vi "Add Files to Project.vi"(8 "error in":errorcluster, 11 "Runner in":refnum<class "Runner.lvclass">) -> (0 "error out":errorcluster, 3 "Runner out":refnum<class "Runner.lvclass">)   [LabVIEW 2026, in "Runner.lvlib" / "Runner.lvclass"]
doc: "This method adds all created files (VIs and Type Definitions) to the project."
uses:
  Runner.lvclass
  Runner.lvclass/Runner.ctl
  Interfaces/ILogger/ILogger Messages/Log Msg/Log Msg.lvclass/Log Msg.ctl
  <vilib>/ActorFramework/Message Enqueuer/Message Enqueuer.lvclass/Message Enqueuer.ctl
  <vilib>/ActorFramework/Message Enqueuer/Enqueue.vi
  Interfaces/ILogger/ILogger Messages/Log Msg/Log Msg.lvclass
  <userlib>/_OpenG.lib/file/file.llb/File Exists - Scalar__ogtk.vi
  <vilib>/ActorFramework/Message Priority Queue/Priority Enqueue.vi
  Interfaces/IProject Manager/IProject Manager.lvclass
  <userlib>/_OpenG.lib/file/file.llb/openg_file.lvlib
  Interfaces/IFile Manager/IFile Manager.lvclass
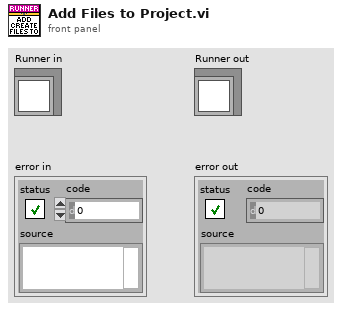
[diagram p1: front panel]
types:
  T1 = typedef "Log Entry--cluster.ctl" = cluster{"Time":timestamp, "Message":string}
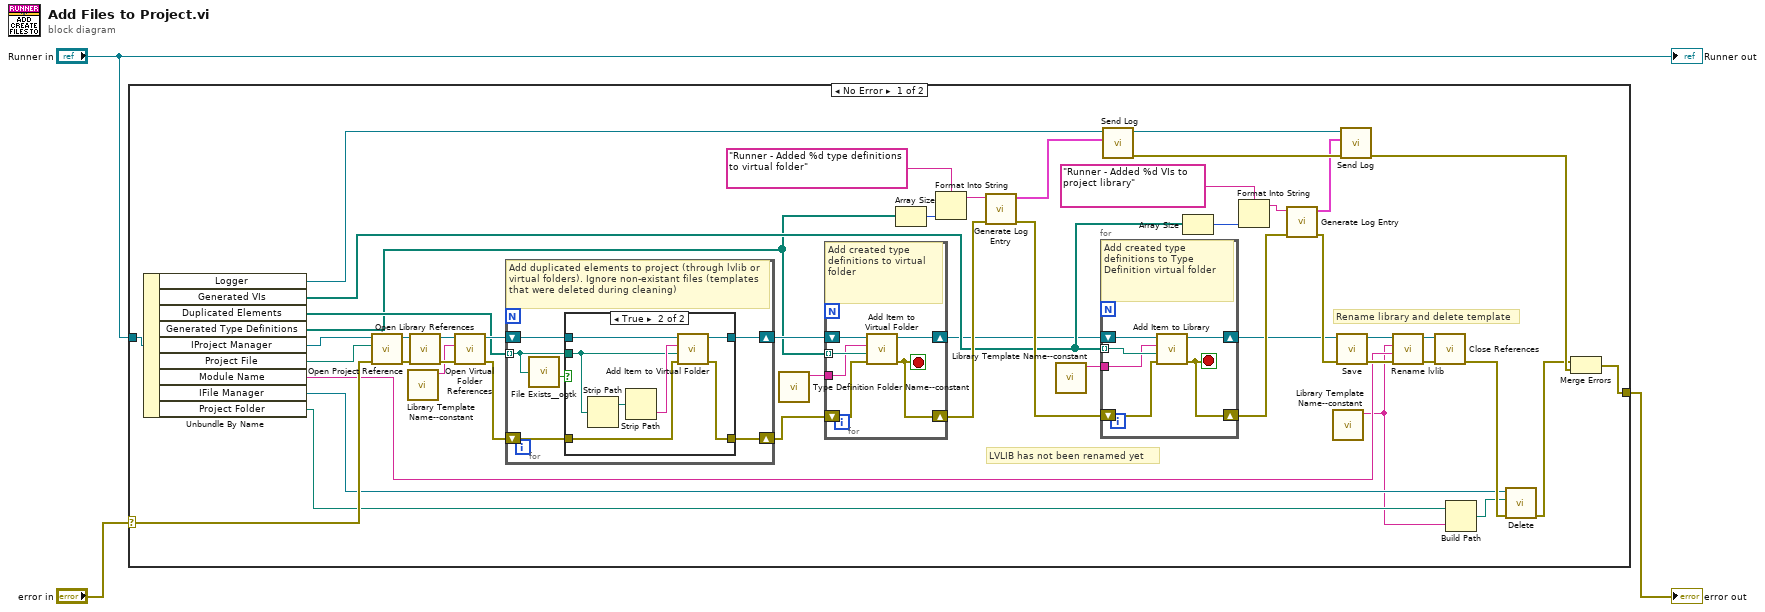
[diagram p0: block diagram]
diagram:
  n1 = case shown="No Error" "error in" {
    selector: "error in" -> [w40 w79]
    tunnel: "Runner in" -> [w35 _]
    tunnel: [w50 w79] -> w2
    frame No Error {
      # "Rename library and delete template"
      # "LVLIB has not been renamed yet"
      n2 = Unbundle By Name(w35) -> ("Logger"=w25:refnum<class "Message Enqueuer.lvclass">, "Generated VIs"=w27:path[], "Duplicated Elements"=w10:path[], "Generated Type Definitions"=w8:path[], "IProject Manager"=w14:refnum<class "IProject Manager.lvclass">, "Project File"=w12:path, "Module Name"=w13:string, "IFile Manager"=w7:refnum<class "IFile Manager.lvclass">, "Project Folder"=w6:path)
      n3 = call-dynamic "Open Project Reference.vi"("error in"=w40, "Path"=w12, "IProject Manager in"=w14) -> ("error out"=w41:errorcluster, "IProject Manager out"=w15:refnum<class "IProject Manager.lvclass">)  [unwired: 7 in]
      n4 = call "Library Template Name--constant.vi"() -> ("Library Template Name"=w17:string)  [unwired: 11 in]
      n5 = call-dynamic "Open Library References.vi"("error in"=w41, "IProject Manager in"=w15) -> ("error out"=w42:errorcluster, "IProject Manager out"=w16:refnum<class "IProject Manager.lvclass">)  [unwired: 8 in]
      n6 = call-dynamic "Open Virtual Folder References.vi"("error in"=w42, "lvlib"=w17, "IProject Manager in"=w16) -> ("error out"=w39:errorcluster, "IProject Manager out"=w11:refnum<class "IProject Manager.lvclass">)  [unwired: 7 in]
      n7 = for {
        tunnel: w10 -> [w53] mode=indexing
        shift-right: [w54] -> w9
        shift-left: w11 -> [w55]
        shift-right: [w56] -> w38
        shift-left: w39 -> [w57]
        # "Add duplicated elements to project (through lvlib or virtual folders). Ignore non-existant files (templates that were deleted during cleaning)"
        n8 = call-poly <userlib>:"File Exists__ogtk.vi"("file path"=w53) -> ("exists"=w52:bool)  [unwired: 6 in, 1 out]
        n9 = case shown="True" w52 {
          tunnel: w57 -> [w59 w66]
          tunnel: [w59 w65] -> w56
          tunnel: w55 -> [w58 w62]
          tunnel: [w58 w61] -> w54
          tunnel: w53 -> [_ w60]
          frame False {
          }
          frame True {
            n10 = Strip Path(path=w60) -> (stripped path=w63:path)  [unwired: 1 out]
            n11 = Strip Path(path=w63) -> (name=w64:string)  [unwired: 1 out]
            n12 = call-dynamic "Add Item to Virtual Folder.vi"("error in"=w66, "File Path"=w60, "Virtual Folder"=w64, "IProject Manager in"=w62) -> ("error out"=w65:errorcluster, "IProject Manager out"=w61:refnum<class "IProject Manager.lvclass">)  [unwired: 6 in]
          }
        }
      }
      n13 = call "Type Definition Folder Name--constant.vi"() -> ("Type Definition Folder Name"=w21:string)  [unwired: 11 in]
      n14 = for {
        tunnel: w8 -> [w74] mode=indexing
        shift-right: [w77] -> w47
        shift-left: w38 -> [w78]
        tunnel: w21 -> [w73]
        shift-right: [w75] -> w23
        shift-left: w9 -> [w76]
        stop <- w77 stop-if-true
        # "Add created type definitions to virtual folder"
        n15 = call-dynamic "Add Item to Virtual Folder.vi"("error in"=w78, "File Path"=w74, "Virtual Folder"=w73, "IProject Manager in"=w76) -> ("error out"=w77:errorcluster, "IProject Manager out"=w75:refnum<class "IProject Manager.lvclass">)  [unwired: 6 in]
      }
      n16 = Array Size(array=w8) -> (size(s)=w32:i32)
      n17 = Format Into String(format string="Runner - Added %d type definitions to virtual folder", w32) -> (resulting string=w31:string)  [unwired: 2 in, 1 out]
      n18 = call "Generate Log Entry.vi"("error in"=w47, "Message"=w31) -> ("error out"=w49:errorcluster, "Log Entry"=w34:T1)  [unwired: 8 in]
      n19 = call "Library Template Name--constant.vi"() -> ("Library Template Name"=w20:string)  [unwired: 11 in]
      n20 = for {
        shift-right: [w71] -> w51
        shift-left: w49 -> [w72]
        tunnel: w27 -> [w68] mode=indexing
        tunnel: w20 -> [w67]
        shift-right: [w69] -> w22
        shift-left: w23 -> [w70]
        stop <- w71 stop-if-true
        # "Add created type definitions to Type Definition virtual folder"
        n21 = call-dynamic "Add Item to Library.vi"("error in"=w72, "Item Path"=w68, "Library"=w67, "IProject Manager in"=w70) -> ("error out"=w71:errorcluster, "IProject Manager out"=w69:refnum<class "IProject Manager.lvclass">)  [unwired: 6 in]
      }
      n22 = call "Send Log.vi"("Log Entry"=w34, "Message Enqueuer"=w25) -> ("error out"=w48:errorcluster, "Message Enqueuer out"=w24:refnum<class "Message Enqueuer.lvclass">)  [unwired: 8 in]
      n23 = Array Size(array=w27) -> (size(s)=w28:i32)
      n24 = Format Into String(format string="Runner - Added %d VIs to project library", w28) -> (resulting string=w26:string)  [unwired: 2 in, 1 out]
      n25 = call "Generate Log Entry.vi"("error in"=w51, "Message"=w26) -> ("error out"=w45:errorcluster, "Log Entry"=w30:T1)  [unwired: 8 in]
      n26 = call "Library Template Name--constant.vi"() -> ("Library Template Name"=w5:string)  [unwired: 11 in]
      n27 = call-dynamic "Save.vi"("error in"=w45, "IProject Manager in"=w22) -> ("error out"=w44:errorcluster, "IProject Manager out"=w19:refnum<class "IProject Manager.lvclass">)  [unwired: 8 in]
      n28 = call "Send Log.vi"("error in (no error)"=w48, "Log Entry"=w30, "Message Enqueuer"=w24) -> ("error out"=w46:errorcluster)  [unwired: 7 in, 1 out]
      n29 = call-dynamic "Rename lvlib.vi"("error in"=w44, "New Name"=w13, "Library"=w5, "IProject Manager in"=w19) -> ("error out"=w43:errorcluster, "IProject Manager out"=w18:refnum<class "IProject Manager.lvclass">)  [unwired: 6 in]
      n30 = call-dynamic "Close References.vi"("error in"=w43, "IProject Manager in"=w18) -> ("error out"=w37:errorcluster)  [unwired: 8 in, 1 out]
      n31 = Build Path(base path=w6, name or relative path=w5) -> (appended path=w4:path)
      n32 = call-dynamic "Delete.vi"("error in"=w37, "Path"=w4, "IFile Manager in"=w7) -> ("error out"=w36:errorcluster)  [unwired: 7 in, 1 out]
      n33 = Merge Errors(w36, w46) -> (w50:errorcluster)
    }
    frame Error {
      # "Pass error without further action."
    }
  }
  "error out" <- w2
  "Runner out" <- "Runner in"
